vi "Read Save Path.vi"(8 "error in (no error)":errorcluster, 11 "Abstract DAQ Triggered Actor in":refnum<class "Abstract DAQ Triggered Actor.lvclass">) -> (0 "error out":errorcluster, 2 "Save Path":path, 3 "Abstract DAQ Triggered Actor out":refnum<class "Abstract DAQ Triggered Actor.lvclass">)   [LabVIEW 2020, in "DAQ Timed SPIM.lvlib" / "Abstract DAQ Triggered Actor.lvlib" / "Abstract DAQ Triggered Actor.lvclass"]
uses:
  Abstract DAQ Triggered Actor.lvclass
  Abstract DAQ Triggered Actor.lvclass/Abstract DAQ Triggered Actor.ctl
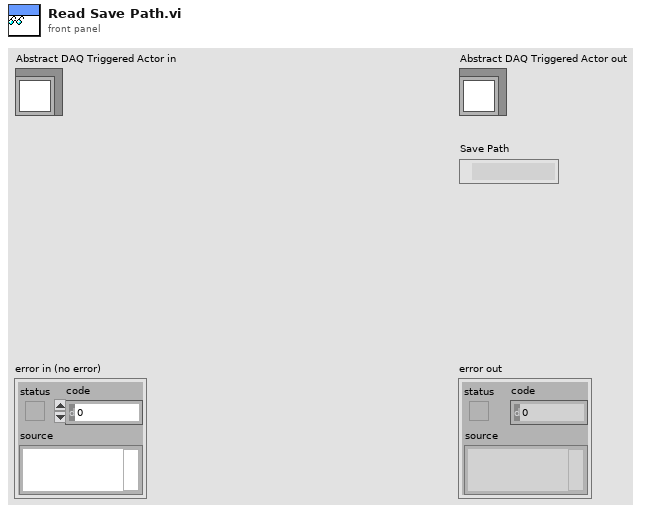
[diagram p1: front panel]
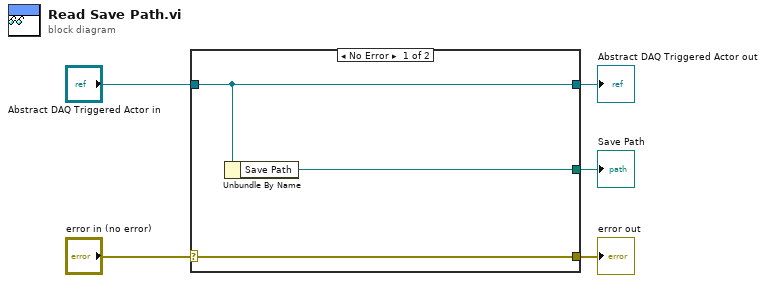
[diagram p0: block diagram]
diagram:
  n1 = case shown="No Error" "error in (no error)" {
    selector: "error in (no error)" -> [w8 w9]
    tunnel: [w8 w9] -> w4
    tunnel: [w7 w10] -> w2
    tunnel: "Abstract DAQ Triggered Actor in" -> [w7 w10]
    tunnel: [w6 _] -> w1
    frame No Error {
      n2 = Unbundle By Name(w7) -> ("Save Path"=w6:path)
    }
    frame Error {
    }
  }
  "error out" <- w4
  "Abstract DAQ Triggered Actor out" <- w2
  "Save Path" <- w1
